vi "Draw Plot.vi"(8 "error in (no error)":errorcluster caption="错误输入（无错误）", 9 "X坐标轴":T1, 11 "Data Viewer 输入":refnum<class "Data Viewer.lvclass">) -> (0 "error out":errorcluster caption="错误输出", 3 "Data Viewer 输出":refnum<class "Data Viewer.lvclass">)   [LabVIEW 2020, in "Data Viewer.lvlib" / "Data Viewer.lvclass"]
uses:
  Data Viewer.lvclass
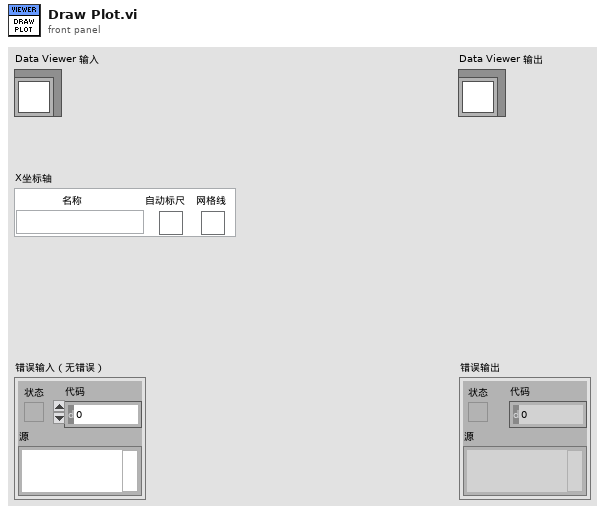
[diagram p1: front panel]
types:
  T1 = cluster{"名称":string, "Auto Scale":bool, "Gird Line":bool}
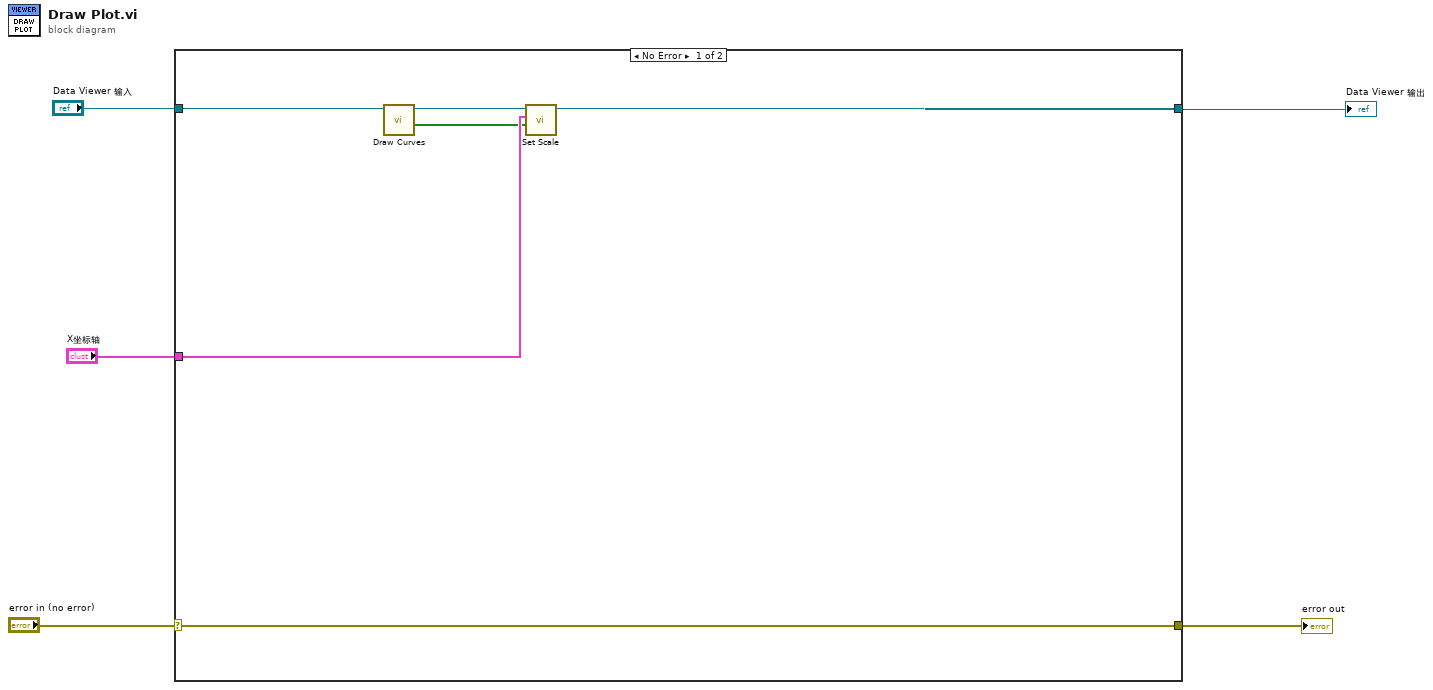
[diagram p0: block diagram]
diagram:
  n1 = case shown="No Error" "error in (no error)" {
    selector: "error in (no error)" -> [w11 w13]
    tunnel: [w11 w13] -> w4
    tunnel: [w7 w12] -> w2
    tunnel: "Data Viewer 输入" -> [w9 w12]
    tunnel: "X坐标轴" -> [w10 _]
    frame No Error {
      n2 = call "Draw Curves.vi"("Data Viewer in"=w9) -> ("Scale Visible"=w6:bool[], "Data Viewer Out"=w8:refnum<class "Data Viewer.lvclass">)  [unwired: 9 in]
      n3 = call "Set Scale.vi"("Scale Visible"=w6, "X坐标轴"=w10, "Data Viewer in"=w8) -> ("Data Viewer Out"=w7:refnum<class "Data Viewer.lvclass">)  [unwired: 8 in]
    }
    frame Error {
    }
  }
  "error out" <- w4
  "Data Viewer 输出" <- w2
